vi "Main.vi"() -> ()   [LabVIEW 2025]
uses:
  <vilib>/Utility/file.llb/Read Delimited Spreadsheet (DBL).vi
  <vilib>/Utility/file.llb/Write Delimited Spreadsheet (I64).vi
panel:
  in  "Neuronal Model":T1(ring)
  in  "Phantom Folder":path
  out "Indentation point number:":i32
  # "Select the file folder and the neuron type:"
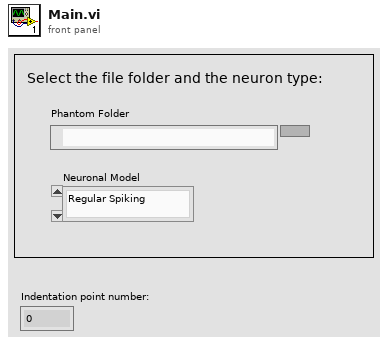
[diagram p1: front panel]
types:
  T1 = enum16{"Regular Spiking", "Chattering", "Fast Spiking"}
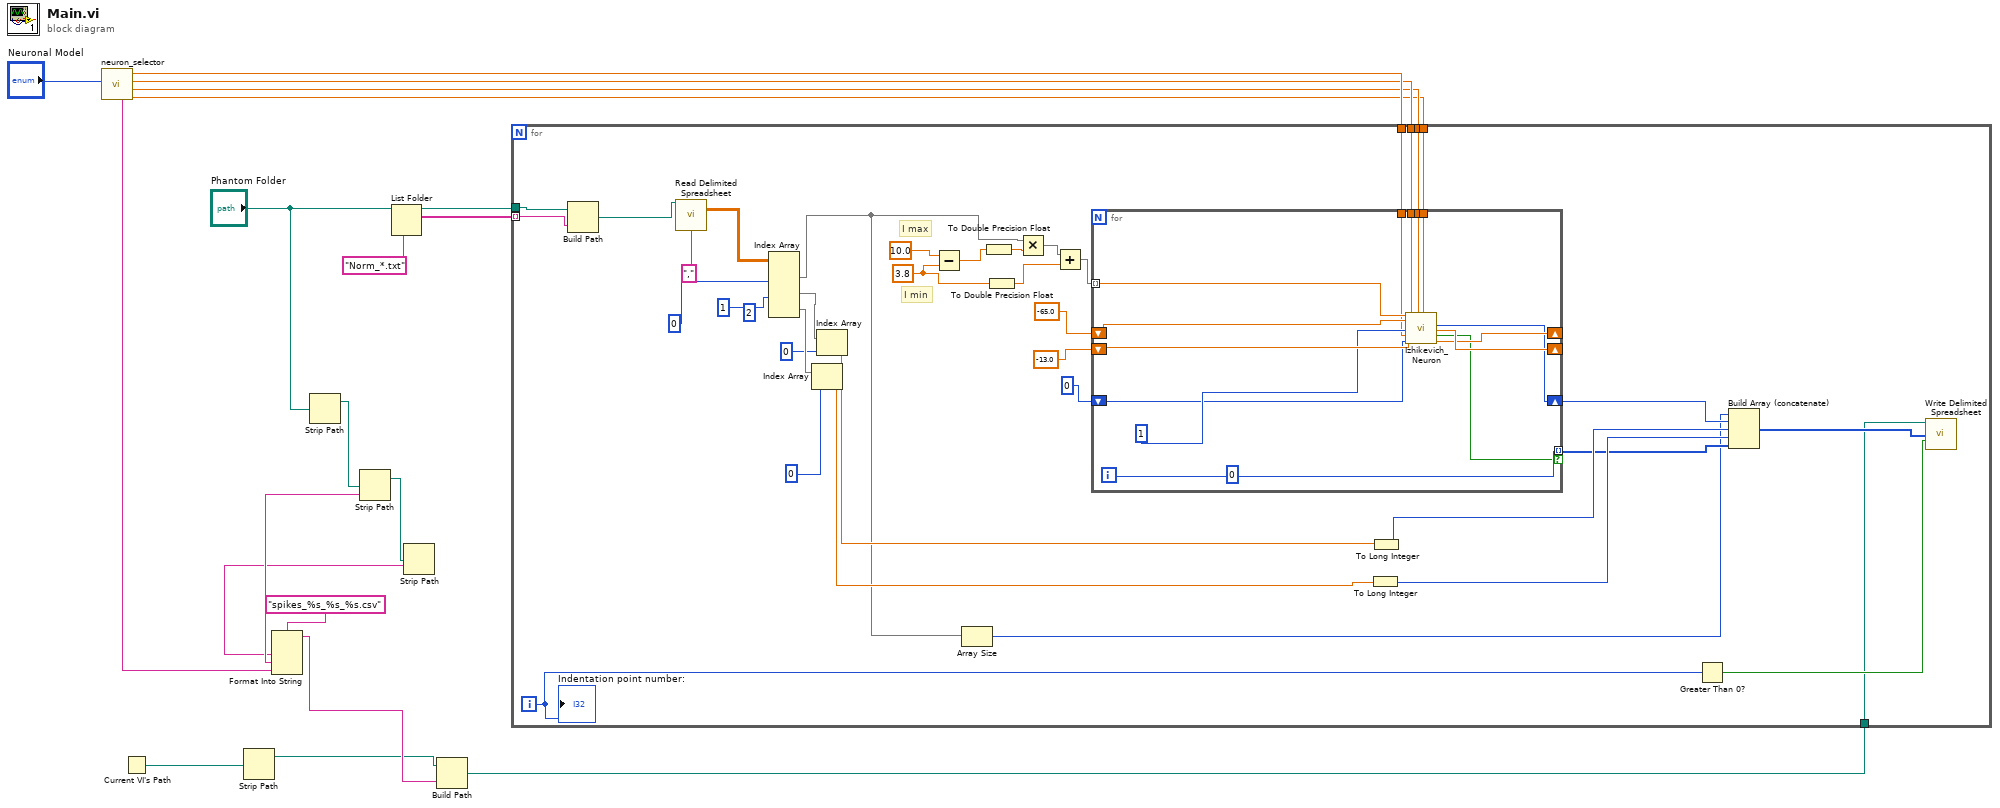
[diagram p0: block diagram]
diagram:
  n1 = call "neuron_selector.vi"("Neuronal Model"="Neuronal Model") -> ("d"=w3:dbl, "c"=w4:dbl, "b"=w5:dbl, "a"=w6:dbl, "Model"=w2:string)  [unwired: 6 in]
  n2 = Current VI's Path() -> (path=w8:path)
  n3 = Strip Path(path=w8) -> (stripped path=w7:path)  [unwired: 1 out]
  n4 = Strip Path(path="Phantom Folder") -> (stripped path=w15:path)  [unwired: 1 out]
  n5 = Strip Path(path=w15) -> (stripped path=w14:path, name=w13:string)
  n6 = List Folder(path="Phantom Folder", pattern="Norm_*.txt") -> (path out=w17:path, filenames=w18:string[])  [unwired: 2 in, 2 out]
  n7 = Strip Path(path=w14) -> (name=w12:string)  [unwired: 1 out]
  n8 = Format Into String(format string="spikes_%s_%s_%s.csv", w12, w13, w2) -> (resulting string=w10:string)  [unwired: 2 in, 1 out]
  n9 = Build Path(base path=w7, name or relative path=w10) -> (appended path=w9:path)
  n10 = for {
    tunnel: w18 -> [w56] mode=indexing
    tunnel: w17 -> [w25]
    tunnel: w9 -> [w24]
    tunnel: w6 -> [w23]
    tunnel: w5 -> [w22]
    tunnel: w4 -> [w21]
    tunnel: w3 -> [w20]
    i -> [w31]
    w42 = 3.8
    (unwired) 0 ("Spike Count Out")
    (unwired) 2 ("index")
    # "I max"
    # "I min"
    n11 = Build Path(base path=w25, name or relative path=w56) -> (appended path=w55:path)
    n12 = call-poly <vilib>:"Read Delimited Spreadsheet.vi"("file path (dialog if empty)"=w55, "delimiter (\\t)"="," ("delimiter (\\t)")) -> ("all rows"=w53:dbl[][])  [unwired: 8 in, 5 out]
    n13 = Index Array(array=w53, index (col) #1=0 ("index (row)"), index (col) #2=1 ("index")) -> (element #1=w27:dbl[], element #2=w49:dbl[], element #3=w52:dbl[])  [unwired: 4 in]
    n14 = Index Array(array=w52, index=0) -> (element=w38:dbl)
    n15 = Index Array(array=w49, index=0) -> (element=w39:dbl)
    n16 = Subtract(x=10.0, y=w42) -> (x-y=w46:dbl)
    n17 = Array Size(array=w27) -> (size(s)=w26:i32)
    n18 = To Double Precision Float(number=w46) -> (double precision float=w45:dbl)
    n19 = To Double Precision Float(number=w42) -> (double precision float=w43:dbl)
    n20 = Multiply(x=w27, y=w45) -> (x*y=w44:dbl[])
    n21 = Add(x=w44, y=w43) -> (x+y=w41:dbl[])
    n22 = for {
      shift-right: [w66] -> _
      shift-left: -65.0 ("v(t+1)") -> [w64]
      shift-right: [w70] -> _
      shift-left: -13.0 ("u(t+1)") -> [w69]
      tunnel: w41 -> [w68] mode=indexing
      tunnel: [w65] -> w29 mode=indexing if=w57
      shift-right: [w62] -> w28
      shift-left: 0 ("Spike Count Out") -> [w63]
      tunnel: w23 -> [w61]
      tunnel: w22 -> [w60]
      tunnel: w21 -> [w59]
      tunnel: w20 -> [w58]
      i -> [w65]
      n23 = call "Izhikevich_Neuron.vi"("I"=w68, "v(t)"=w64, "u(t)"=w69, "dt"=u32 1 ("millisecond multiple"), "a"=w61, "Spike Count In"=w63, "b"=w60, "c"=w59, "d"=w58) -> ("Spike Count Out"=w62:i32, "u(t+dt)"=w70:dbl, "Spike detected"=w57:bool, "v(t+dt)"=w66:dbl)  [unwired: 7 in]
    }
    n24 = To Long Integer(number=w38) -> (32bit integer=w34:i32)
    n25 = To Long Integer(number=w39) -> (32bit integer=w35:i32)
    n26 = Greater Than 0?(x=w31) -> (x > 0?=w33:bool)
    n27 = Build Array (concatenate)(w26, w28, w35, w34, w29) -> (w32:i32[])
    n28 = call-poly <vilib>:"Write Delimited Spreadsheet.vi"("file path (dialog if empty)"=w24, "1D data"=w32, "append to file? (new file:F)"=w33) -> ()  [unwired: 11 in, 2 out]
    "Indentation point number:" <- w31
  }
